vi "mupExpr sglExpr multiVar example.vi"() -> ()   [LabVIEW 2015]
uses:
  mupExpr/mupExpr.lvclass
  mupExpr/mupExpr.lvclass/mupExpr.ctl
  mupExpr/Eval_MultiVar_SglRes.vi
  mupExpr/SetVarVal.vi
  mupLib/mupEval.vi
  mupLib/mupSetVarValue.vi
  mupLib/mupCheckError.vi
  mupLib/mupLibPath.vi
  <vilib>/Utility/error.llb/Error Cluster From Error Code.vi
panel:
  out "error out":errorcluster
  out "Result":dbl format="%#_13g"
  out "Variable Names":string[](array[string])
  in  "Expression":string="sin(w*t+c)"
  in  "Variable Values":dbl[](array[numeric])=[0.0, 1.0, 3.141592654] format="%#_13g"
  # "This example demonstrates the evaluation of a multi-variable expression.\n\n- Enter an expression composed of any number of variables\n- Enter the value of each variable (variables are listed in alphabetical order)\n- Hit run to evaluate the expression"
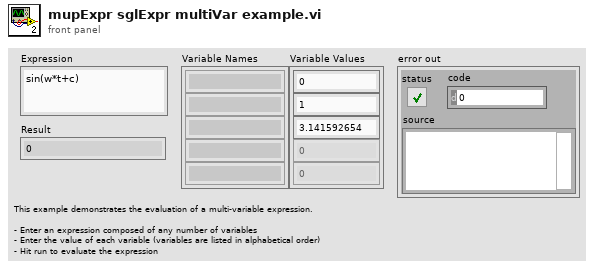
[diagram p1: front panel]
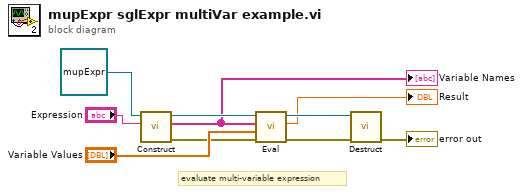
[diagram p0: block diagram]
diagram:
  # "evaluate multi-variable expression"
  n1 = call-dynamic "Construct.vi"("Expression"="Expression", "muExpr in"=refnum<class "mupExpr.lvclass"> refnum) -> ("error out"=w4:errorcluster, "Variable Names"=w6:string[], "mupExpr out"=w8:refnum<class "mupExpr.lvclass">)  [unwired: 6 in, 1 out]
  "Variable Names" <- w6
  n2 = call-poly "Eval.vi"("error in (no error)"=w4, "varValues"="Variable Values", "varNames"=w6, "muExpr in"=w8) -> ("error out"=w3:errorcluster, "Result"=→"Result":dbl, "muExpr out"=w7:refnum<class "mupExpr.lvclass">)  [unwired: 5 in]
  n3 = call-dynamic "Destruct.vi"("error in (no error)"=w3, "muExpr in"=w7) -> ("error out"=→"error out":errorcluster)  [unwired: 9 in]
